vi "Demo 1-clon.vi"() -> ()   [LabVIEW 2026]
panel:
  out "Waveform Chart":dbl(graph)
  out "Gauge":dbl(knob) scale=0.0..10.0
  in  "Numeric":dbl
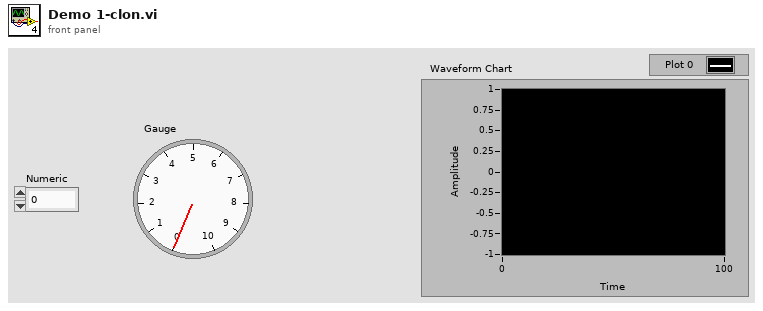
[diagram p1: front panel]
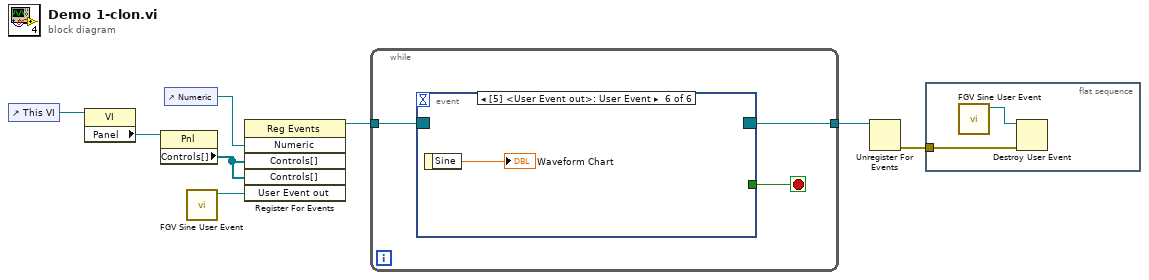
[diagram p0: block diagram]
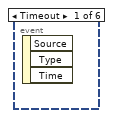
[diagram p2: hidden frame]
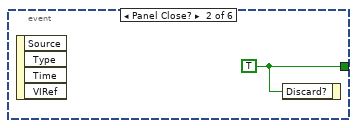
[diagram p3: hidden frame]
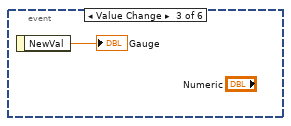
[diagram p4: hidden frame]
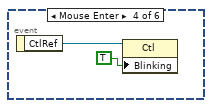
[diagram p5: hidden frame]
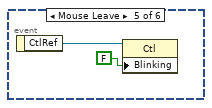
[diagram p6: hidden frame]
diagram:
  n1 = control-ref of="This VI"() -> (w4:refnum<vi>)
  n2 = property class="VI"(reference=w4) -> ("Panel"=w3:refnum<vi>)  [unwired: 1 in, 2 out]
  n3 = property class="Pnl"(reference=w3) -> ("Controls[]"=w2:refnum<vi>[])  [unwired: 1 in, 2 out]
  n4 = control-ref of="Numeric"() -> (w5:refnum<vi>)
  n5 = call "FGV Sine User Event.vi"() -> ("User Event out"=w1:refnum<user-event>)  [unwired: 10 in, 1 out]
  n6 = register-events(w5, w2, w2, w1) -> (reference out=w7:refnum<event-registration>)  [unwired: 2 in, 1 out]
  n7 = while {
    tunnel: w7 -> [w10]
    tunnel: [w9] -> w6
    stop <- w11 stop-if-true
    n8 = event shown="[5] <User Event out>: User Event" {
      selector: w10 -> [_ _ _ _ _ _]
      dyn-events: [_ _ _ _ _ _] -> w9
      timeout: _ -> [_ _ _ _ _ _]
      tunnel: [_ w12 _ _ _ _] -> w11
      event Timeout {
        n9 = event-data() -> ()  [unwired: 1 in, 3 out]
      }
      event Panel Close? {
        w12 = TRUE ("Discard?")
        n10 = event-data() -> ()  [unwired: 1 in, 4 out]
        n11 = event-data("Discard?"=w12) -> ()  [unwired: 1 in, 1 out]
      }
      event Value Change {
        n12 = event-data() -> ("NewVal"=→"Gauge":dbl)  [unwired: 1 in]
      }
      event Mouse Enter {
        n13 = event-data() -> ("CtlRef"=w15:refnum<vi>)  [unwired: 1 in]
        n14 = property class="Ctl"(reference=w15, "Blinking"=TRUE) -> ()  [unwired: 1 in, 2 out]
      }
      event Mouse Leave {
        n15 = event-data() -> ("CtlRef"=w17:refnum<vi>)  [unwired: 1 in]
        n16 = property class="Ctl"(reference=w17, "Blinking"=FALSE) -> ()  [unwired: 1 in, 2 out]
      }
      event User Event {
        n17 = event-data() -> ("Sine"=→"Waveform Chart":dbl)  [unwired: 1 in]
      }
    }
  }
  n18 = Unregister For Events(event registration refnum=w6) -> (error out=w8:errorcluster)  [unwired: 1 in]
  n19 = flat-sequence {
    tunnel: w8 -> [w20]
    frame #0 {
      n20 = call "FGV Sine User Event.vi"() -> ("User Event out"=w19:refnum<user-event>)  [unwired: 10 in, 1 out]
      n21 = Destroy User Event(user event=w19, error in=w20) -> ()  [unwired: 1 out]
    }
  }
